vi "Offline valve lamp.vi"(0 "Position word":u32, 1 "Bit offset":u32, 2 "Physical selectors":u32, 3 "Selector quality":u32) -> (15 "Lamp":picture)   [LabVIEW 2025]
doc: "Render valve position. Grey means unavailable or between endpoints."
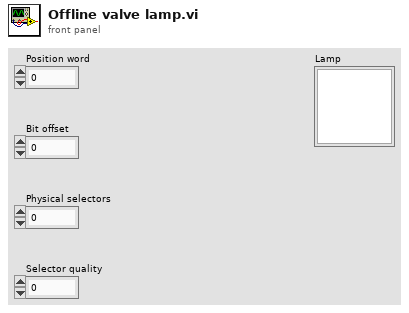
[diagram p1: front panel]
types:
  T1 = cluster{"left":i16, "top":i16, "right":i16, "bottom":i16}
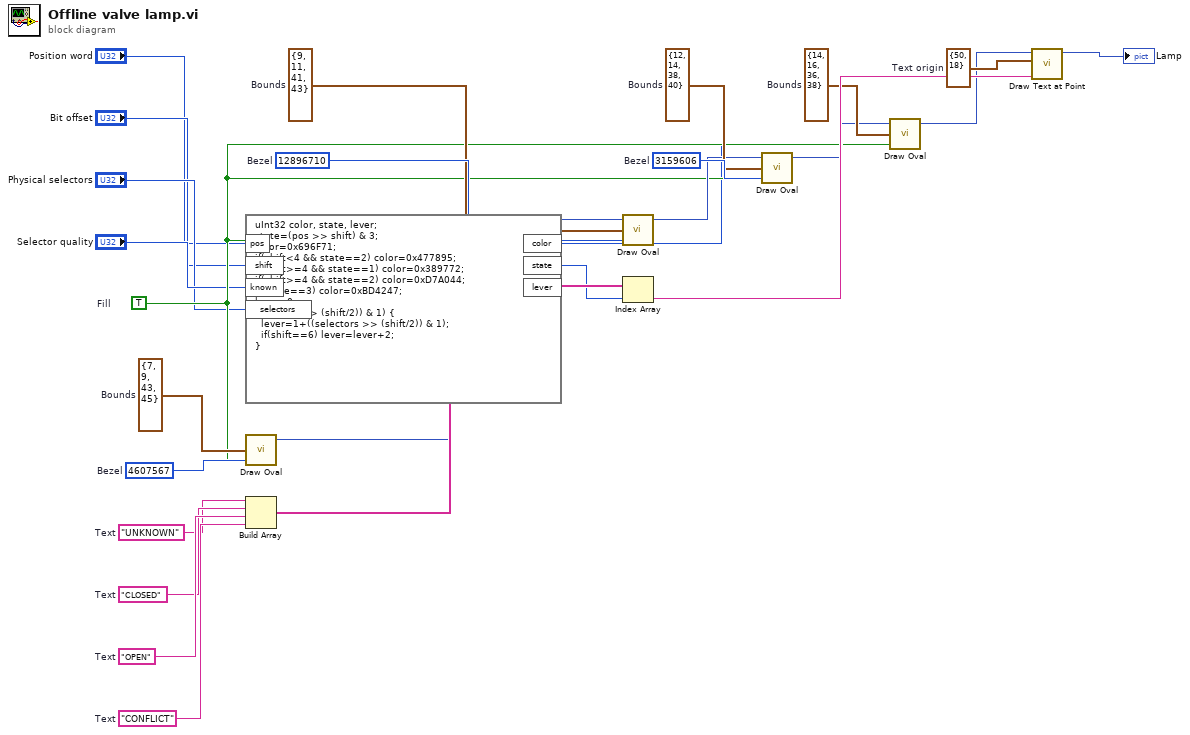
[diagram p0: block diagram]
diagram:
  w25 = cluster{"x":i16, "y":i16} {"x"=50, "y"=18}  # Text origin
  w22 = "CONFLICT"  # Text
  w21 = "OPEN"  # Text
  w20 = "CLOSED"  # Text
  w19 = "UNKNOWN"  # Text
  w17 = T1 {"left"=14, "top"=16, "right"=36, "bottom"=38}  # Bounds
  w15 = u32 3159606  # Bezel
  w14 = T1 {"left"=12, "top"=14, "right"=38, "bottom"=40}  # Bounds
  w12 = u32 12896710  # Bezel
  w11 = T1 {"left"=9, "top"=11, "right"=41, "bottom"=43}  # Bounds
  w9 = u32 4607567  # Bezel
  w8 = T1 {"left"=7, "top"=9, "right"=43, "bottom"=45}  # Bounds
  w7 = TRUE  # Fill
  n1 = formula code="uInt32 color, state, lever;\nstate=(pos >> shift) & 3;\ncolor=0x696F71;\nif(shift<4 && state==2) color=0x477895;\nif(shift>=4 && state==1) color=0x389772;\nif(shift>=4 && state==2) color=0xD7A044;\nif(state==3) color=0xBD4247;\nlever=0;\nif((known >> (shift/2)) & 1) {\n  lever=1+((selectors >> (shift/2)) & 1);\n  if(shift==6) lever=lever+2;\n}"("pos"="Position word", "shift"="Bit offset", "known"="Selector quality", "selectors"="Physical selectors") -> ("color"=w5:u32, "state"=w6:u32)  [unwired: 1 out]
  n2 = call <vilib>:"Draw Oval.vi"("rect"=w8, "fill?(F)"=w7, "color(black)"=w9) -> ("new picture"=w10:picture)  [unwired: 6 in]
  n3 = Build Array(w19, w20, w21, w22) -> (w23:string[])
  n4 = call <vilib>:"Draw Oval.vi"("picture"=w10, "rect"=w11, "fill?(F)"=w7, "color(black)"=w12) -> ("new picture"=w13:picture)  [unwired: 5 in]
  n5 = Index Array(array=w23, index=w6) -> (element=w24:string)
  n6 = call <vilib>:"Draw Oval.vi"("picture"=w13, "rect"=w14, "fill?(F)"=w7, "color(black)"=w15) -> ("new picture"=w16:picture)  [unwired: 5 in]
  n7 = call <vilib>:"Draw Oval.vi"("picture"=w16, "rect"=w17, "fill?(F)"=w7, "color(black)"=w5) -> ("new picture"=w18:picture)  [unwired: 5 in]
  n8 = call <vilib>:"Draw Text at Point.vi"("text"=w24, "origin"=w25, "picture"=w18) -> ("new picture"=→"Lamp":picture)  [unwired: 7 in, 1 out]
